vi "Add User to Group.vi"(5 "Save File":bool=TRUE, 6 "error in (no error)":errorcluster, 7 "Group Name":string, 8 "LoginName":string, 9 "EasyUserManager in":refnum<class "EasyUserManager.lvclass">) -> (0 "error out":errorcluster, 3 "EasyUserManager out":refnum<class "EasyUserManager.lvclass">)   [LabVIEW 2024, in "EasyUserManager.lvclass"]
doc: "Add the user specified by <B>LoginName</B> to the group specified by <B>Group Name</B>. \n\nThe boolean input <B>Save File</B> controls whether changes are immediately saved to the users file (Default: True)."
uses:
  EasyUserManager.lvclass
  EasyUserManager.lvclass/EasyUserManager.ctl
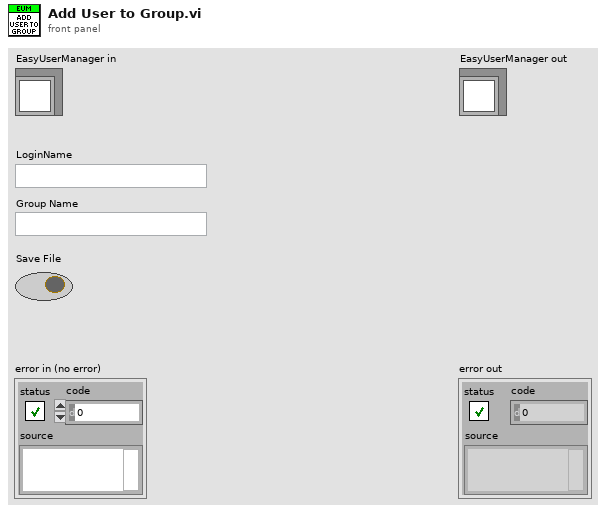
[diagram p1: front panel]
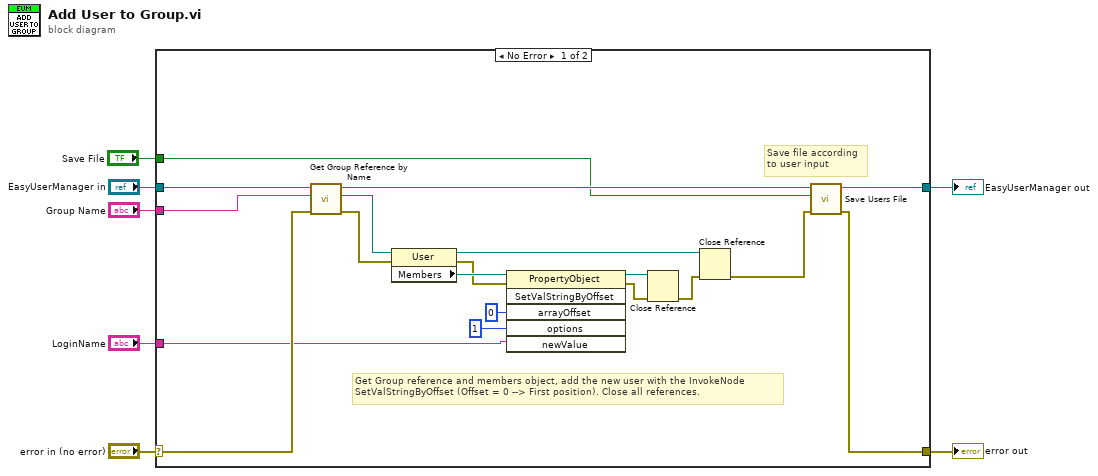
[diagram p0: block diagram]
diagram:
  n1 = case shown="No Error" "error in (no error)" {
    selector: "error in (no error)" -> [w11 w28]
    tunnel: [w25 w28] -> w6
    tunnel: [w26 w27] -> w4
    tunnel: "EasyUserManager in" -> [w23 w27]
    tunnel: "Group Name" -> [w10 _]
    tunnel: "LoginName" -> [w9 _]
    tunnel: "Save File" -> [w8 _]
    frame No Error {
      # "Get Group reference and members object, add the new user with the InvokeNode\nSetValStringByOffset (Offset = 0 --> First position). Close all references."
      # "Save file according\nto user input"
      n2 = call "Get Group Reference by Name.vi"("error in (no error)"=w11, "Group Name"=w10, "EasyUserManager in"=w23) -> ("error out"=w13:errorcluster, "Group Reference"=w14:refnum<k7>, "EasyUserManager out"=w24:refnum<class "EasyUserManager.lvclass">)  [unwired: 2 in]
      n3 = property on="Property Node" class="User"(reference=w14, error in=w13) -> (reference out=w15:refnum<k7>, error out=w21:errorcluster, "Members"=w22:refnum<k7>)
      n4 = invoke on="Invoke Node" class="PropertyObject" method="SetValStringByOffset"(reference=w22, error in=w21, "arrayOffset"=0, "options"=1, "newValue"=w9) -> (reference out=w18:refnum<k7>, error out=w17:errorcluster)  [unwired: 1 in, 4 out]
      n5 = Close Reference(reference=w18, error in (no error)=w17) -> (error out=w16:errorcluster)
      n6 = Close Reference(reference=w15, error in (no error)=w16) -> (error out=w12:errorcluster)
      n7 = call "Save Users File.vi"("error in (no error)"=w12, "Save"=w8, "EasyUserManager in"=w24) -> ("error out"=w25:errorcluster, "EasyUserManager out"=w26:refnum<class "EasyUserManager.lvclass">)  [unwired: 3 in]
    }
    frame Error {
      # "Pass error and do nothing."
    }
  }
  "error out" <- w6
  "EasyUserManager out" <- w4
